vi "power.vi"(8 "error in (no error)":errorcluster, 11 "BasicRemote in":refnum<class "BasicRemote.lvclass">) -> (0 "error out":errorcluster, 3 "BasicRemote out":refnum<class "BasicRemote.lvclass">)   [LabVIEW 2018, in "BasicRemote.lvclass"]
uses:
  BasicRemote.lvclass
  ConsoleOut/Print Options.ctl
  Device Class/Device.lvclass
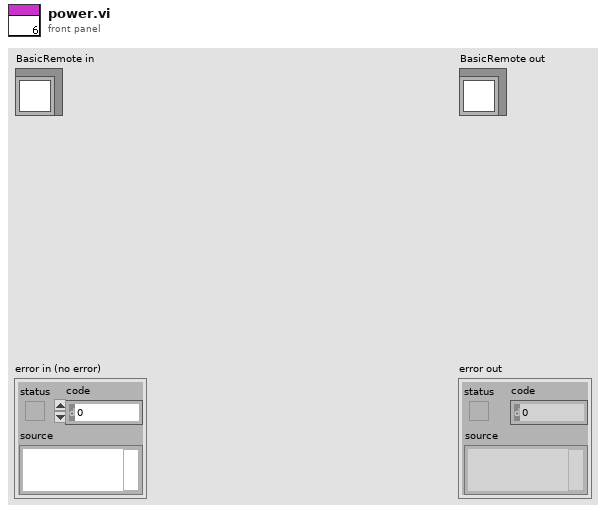
[diagram p1: front panel]
types:
  T1 = typedef "Print Options.ctl" = enum16{"Create", "Get Reference", "Print", "Print Header", "Close"}
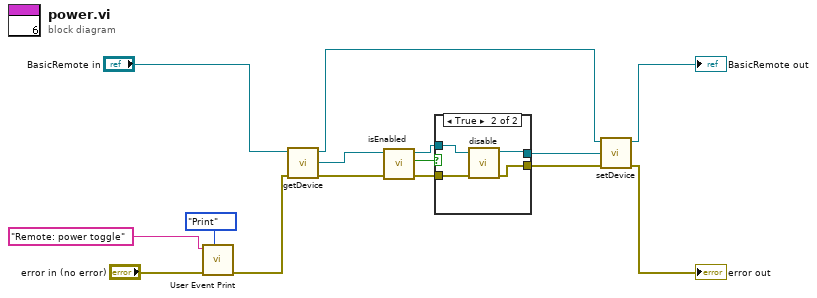
[diagram p0: block diagram]
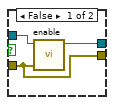
[diagram p2: hidden frame]
diagram:
  n1 = call "User Event Print.vi"("Options"=Print_Options."Print", "error in (no error)"="error in (no error)", "String to Print"="Remote: power toggle" ("message")) -> ("error out"=w4:errorcluster)  [unwired: 7 in, 1 out]
  n2 = call-dynamic "getDevice.vi"("error in (no error)"=w4, "BasicRemote in"="BasicRemote in") -> ("error out"=w3:errorcluster, "Device.lvclass"=w13:refnum<class "Device.lvclass">, "BasicRemote out"=w8:refnum<class "BasicRemote.lvclass">)  [unwired: 7 in]
  n3 = call-dynamic "isEnabled.vi"("error in (no error)"=w3, "Device in"=w13) -> ("error out"=w10:errorcluster, "on"=w12:bool, "Device out"=w11:refnum<class "Device.lvclass">)  [unwired: 7 in]
  n4 = case shown="True" w12 {
    tunnel: w11 -> [w18 w22]
    tunnel: w10 -> [w17 w21]
    tunnel: [w16 w20] -> w9
    tunnel: [w17 w19] -> w2
    frame False {
      n5 = call-dynamic "enable.vi"("error in (no error)"=w17, "Device in"=w18) -> ("Device out"=w16:refnum<class "Device.lvclass">)  [unwired: 8 in, 1 out]
    }
    frame True {
      n6 = call-dynamic "disable.vi"("error in (no error)"=w21, "Device in"=w22) -> ("error out"=w19:errorcluster, "Device out"=w20:refnum<class "Device.lvclass">)  [unwired: 8 in]
    }
  }
  n7 = call-dynamic "setDevice.vi"("error in (no error)"=w2, "Device.lvclass"=w9, "BasicRemote in"=w8) -> ("error out"=→"error out":errorcluster, "BasicRemote out"=→"BasicRemote out":refnum<class "BasicRemote.lvclass">)  [unwired: 7 in]
